vi "Cleanup.vi"(8 "error in (no error)":errorcluster, 11 "SolutionBuilder in":refnum<class "SolutionBuilder.lvclass">) -> (0 "error out":errorcluster, 3 "SolutionBuilder out":refnum<class "SolutionBuilder.lvclass">)   [LabVIEW 2019, in "SolutionBuilder.lvlib" / "SolutionBuilder.lvclass"]
uses:
  SolutionBuilder.lvclass
  SolutionBuilder.lvclass/SolutionBuilder.ctl
  Private/ProjectItemMap.ctl
  ProjectItem/ProjectItem.lvclass
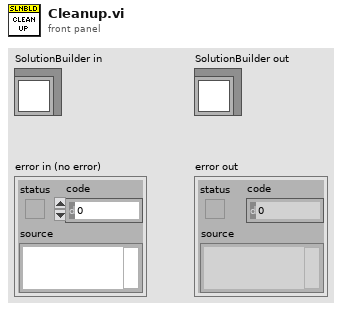
[diagram p1: front panel]
types:
  T1 = typedef "SolutionBuilder.lvlib/SolutionBuilder.lvclass/ProjectItemMap.ctl" = map{path, refnum<class "ProjectItem.lvclass">[]}
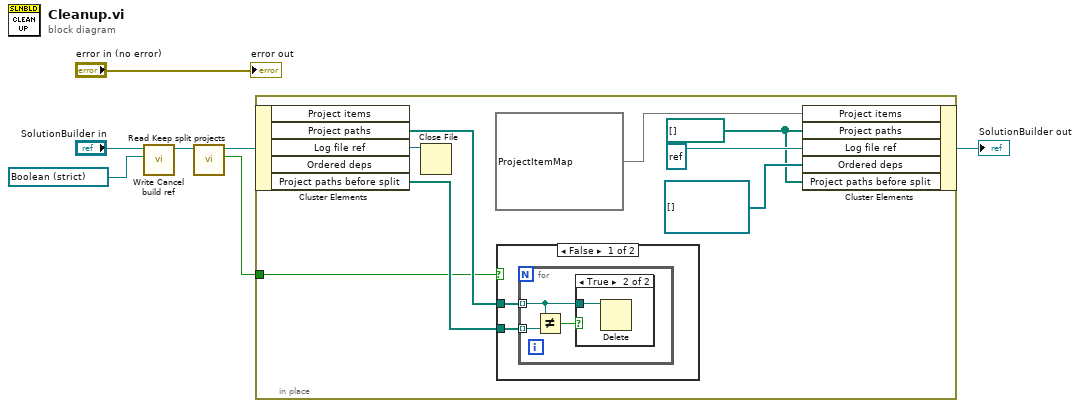
[diagram p0: block diagram]
diagram:
  n1 = call "Write Cancel build ref.vi"("Cancel build ref"=refnum<vi> refnum, "SolutionBuilder in"="SolutionBuilder in") -> ("SolutionBuilder out"=w3:refnum<class "SolutionBuilder.lvclass">)  [unwired: 9 in]
  n2 = call-dynamic "Read Keep split projects.vi"("SolutionBuilder in"=w3) -> ("Keep split projects?"=w1:bool, "SolutionBuilder out"=w2:refnum<class "SolutionBuilder.lvclass">)  [unwired: 9 in]
  n3 = in-place {
    in-place-border: w1 -> [w8]
    w11 = path[] [] ("Project paths")
    n4 = in-place-cluster #1(w2) -> ("Project paths"=w10:path[], "Log file ref"=w13:refnum<file>, "Project paths before split"=w9:path[])  [unwired: 2 out]
    n5 = Close File(refnum=w13) -> ()  [unwired: 1 in, 2 out]
    n6 = case shown="False" w8 {
      tunnel: w10 -> [w17 _]
      tunnel: w9 -> [w16 _]
      frame False {
        n7 = for {
          tunnel: w17 -> [w19] mode=indexing
          tunnel: w16 -> [w20] mode=indexing
          n8 = Not Equal?(x=w19, y=w20) -> (x != y?=w18:bool)
          n9 = case shown="True" w18 {
            tunnel: w19 -> [_ w21]
            frame False {
            }
            frame True {
              n10 = Delete(path (use dialog)=w21) -> ()  [unwired: 4 in, 3 out]
            }
          }
        }
      }
      frame True {
      }
    }
    n11 = in-place-cluster #1("Project items"=T1 {}, "Project paths"=w11, "Log file ref"=refnum<file> refnum, "Ordered deps"=refnum<class "ProjectItem.lvclass">[] [], "Project paths before split"=w11) -> (→"SolutionBuilder out":refnum<class "SolutionBuilder.lvclass">)
  }
  "error out" <- "error in (no error)"
